vi "Get Account.vi"(8 "error in":errorcluster, 10 "Account Number":string, 11 "Accounts File Path":path) -> (0 "error out":errorcluster, 2 "Account":T1, 3 "Account Found?":bool)   [LabVIEW 2026]
doc: "Reads the accounts file and returns the record of one account, so the balance always comes from the file. Account Found? is FALSE with an empty record when the number is not in the file (not an error). Errors of Read Accounts.vi (5001 for an empty path, file errors) are returned in error out; when error in carries an error the file is not read."
uses:
  Controls/ATM Account.ctl
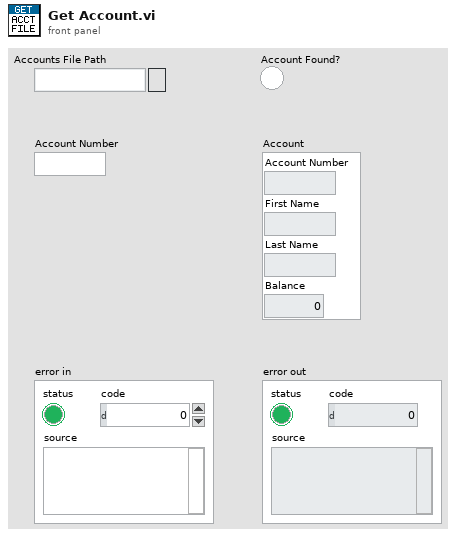
[diagram p1: front panel]
types:
  T1 = typedef "ATM Account.ctl" = cluster{"Account Number":string, "First Name":string, "Last Name":string, "Balance":dbl}
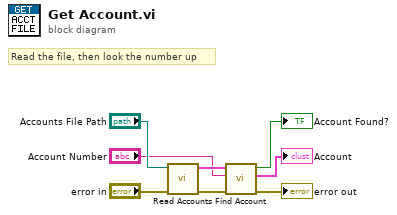
[diagram p0: block diagram]
diagram:
  # "Read the file, then look the number up"
  n1 = call "Read Accounts.vi"("error in"="error in", "Accounts File Path"="Accounts File Path") -> ("error out"=w4:errorcluster, "Accounts"=w6:T1[])  [unwired: 8 in]
  n2 = call "Find Account.vi"("error in"=w4, "Account Number"="Account Number", "Accounts"=w6) -> ("error out"=→"error out":errorcluster, "Account"=→"Account":T1, "Account Found?"=→"Account Found?":bool)  [unwired: 5 in, 1 out]
